vi "Dispose.vi"(8 "error in (no error)":errorcluster, 11 "Navigator in":refnum<class "Navigator.lvclass">) -> (0 "error out":errorcluster, 3 "Navigator out":refnum<class "Navigator.lvclass">)   [LabVIEW 2024, in "Navigator.lvclass"]
doc: "Destroy user events and stop asynchronous event handling loop."
uses:
  Navigator.lvclass
  Navigator.lvclass/Navigator.ctl
  NavigatableView/NavigatableView.lvclass
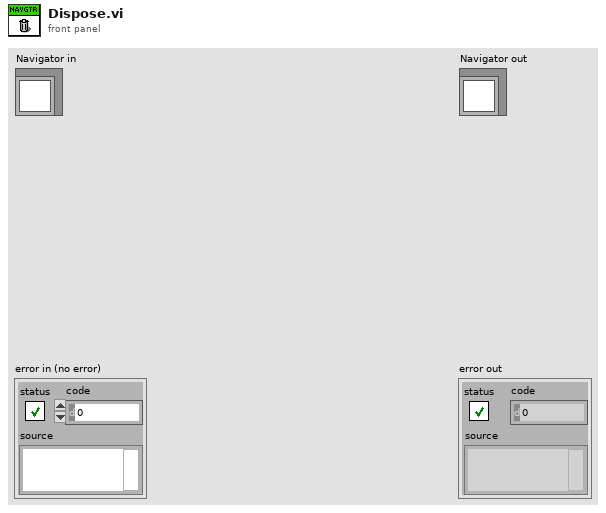
[diagram p1: front panel]
types:
  T1 = typedef "Navigator.lvclass/NavigatorEvents.ctl" = cluster{"go":refnum<user-event>, "push":refnum<user-event>, "pop":refnum<user-event>}
  T2 = typedef "Navigator.lvclass/Route.ctl" = cluster{"Name":string, "Path":path, "Builder":refnum<class "NavigatableView.lvclass">}
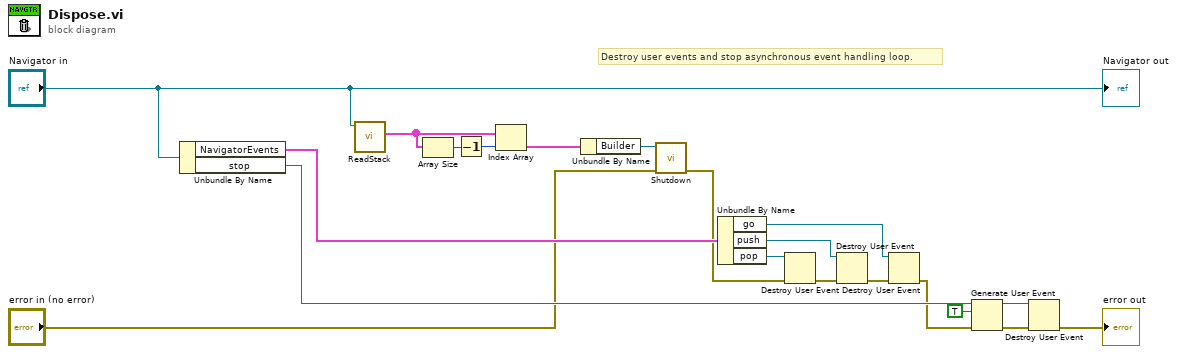
[diagram p0: block diagram]
diagram:
  # "Destroy user events and stop asynchronous event handling loop."
  n1 = Unbundle By Name("Navigator in") -> ("NavigatorEvents"=w16:T1, "stop"=w17:refnum<user-event>)
  n2 = call "ReadStack.vi"("Navigator in"="Navigator in") -> ("Stack"=w2:T2[])  [unwired: 8 in, 2 out]
  n3 = Array Size(array=w2) -> (size(s)=w5:i32)
  n4 = Decrement(x=w5) -> (x-1=w4:i32)
  n5 = Index Array(array=w2, index=w4) -> (element=w1:T2)
  n6 = Unbundle By Name(w1) -> ("Builder"=w3:refnum<class "NavigatableView.lvclass">)
  n7 = call-dynamic "Shutdown.vi"("error in (no error)"="error in (no error)", "NavigatableView in"=w3) -> ("error out"=w7:errorcluster)  [unwired: 8 in, 1 out]
  n8 = Unbundle By Name(w16) -> ("go"=w11:refnum<user-event>, "push"=w12:refnum<user-event>, "pop"=w15:refnum<user-event>)
  n9 = Destroy User Event(user event=w15, error in=w7) -> (error out=w13:errorcluster)
  n10 = Destroy User Event(user event=w12, error in=w13) -> (error out=w14:errorcluster)
  n11 = Destroy User Event(user event=w11, error in=w14) -> (error out=w10:errorcluster)
  n12 = Generate User Event(user event=w17, event data cluster=TRUE ("event data"), error in=w10) -> (user event out=w18:refnum<user-event>, error out=w9:errorcluster)  [unwired: 1 in]
  n13 = Destroy User Event(user event=w18, error in=w9) -> (error out=→"error out":errorcluster)
  "Navigator out" <- "Navigator in"
